vi "Turn Smother.vi"(2 "Ignore Deceleration":bool, 3 "Ignore Acceleration":bool, 4 "Internal Path Stuff":T2={"Trajectory Data"=[], "Updated Waypoints"=[], {"Sample Period (s)"=0.0, "Limits"={"Velocity (fps)"=0.0, "Accel (fps^2)"=0.0, "Jerk (fps^3)"=0.0, "StoopidFast (fps)"=0.0}, "Conditions"={"vInitial (fps)"=0.0, "vFinal (fps)"=0.0}, "Overrides"=[], "Angular Limits"={"Velocity (deg/s)"=6.0, "Accel (deg/s^2)"=15.0, "Jerk (deg/s^3)"=150.0}}, "Commands out"=[]} {"?"."Angular Limits"."Jerk (deg/s^3)" min=0.0 step=1.0; "?"."Angular Limits"."Accel (deg/s^2)" min=0.0; "?"."Angular Limits"."Velocity (deg/s)" min=0.0; "?"."Limits"."StoopidFast (fps)" min=0.0; "?"."Limits"."Jerk (fps^3)" min=0.0 step=1.0; "?"."Limits"."Accel (fps^2)" min=0.0; "?"."Limits"."Velocity (fps)" min=0.0; "?"."Overrides"."Angle Override" step=5.0; "?"."Overrides"."Velocity Override" step=5.0; "?"."Overrides"."Angular Override" step=5.0}) -> (1 "Overrides":T1 {"Angle Override" step=5.0; "Velocity Override" step=5.0; "Angular Override" step=5.0})   [LabVIEW 2023]
uses:
  Types/Internal Path Stuff.ctl
  Types/Trajectory Data.ctl
  Types/Segment Type.ctl
  Types/Limits.ctl
  Types/Overrides.ctl
  Types/Angluar Limits.ctl
  Types/Single Cmd Info.ctl
  <vilib>/picture/picture.llb/imagedata.ctl
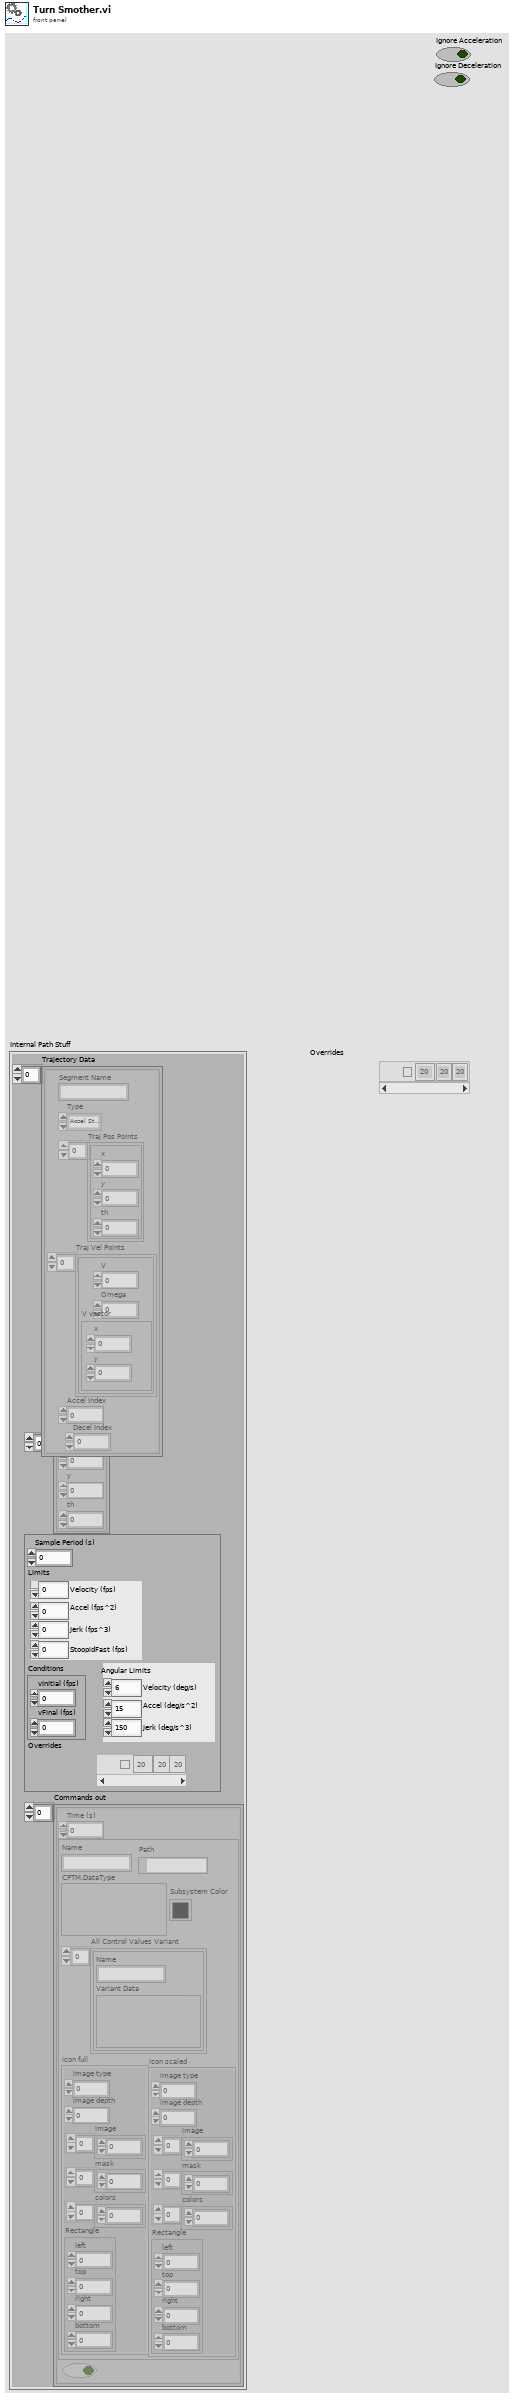
[diagram p1: front panel]
types:
  T1 = typedef "Overrides.ctl" = cluster{"Count":string, "Angular Override":dbl, "Enabled?":bool, "Velocity Override":dbl, "Angle Override":dbl}[]
  T2 = typedef "Internal Path Stuff.ctl" = cluster{"Trajectory Data":T3, "Updated Waypoints":cluster{"x":dbl, "y":dbl, "th":dbl}[], cluster{"Sample Period (s)":dbl, "Limits":T5, "Conditions":cluster{"vInitial (fps)":dbl, "vFinal (fps)":dbl}, "Overrides":T1, "Angular Limits":T6}, "Commands out":cluster{"Time (s)":dbl, T7, bool}[]}
  T3 = typedef "Trajectory Data.ctl" = cluster{"Segment Name":string, "Type":T4, "Traj Pos Points":cluster{"x":dbl, "y":dbl, "th":dbl}[], "Traj Vel Points":cluster{"V":dbl, "Omega":dbl, "V vector":cluster{"y":dbl, "x":dbl}}[], "Accel Index":i32, "Decel Index":i32}[]
  T4 = typedef "Segment Type.ctl" = enum16{"Accel Straight", "Const Straight", "Blend", "Circle", "Bezier"}
  T5 = typedef "Limits.ctl" = cluster{"Velocity (fps)":dbl, "Accel (fps^2)":dbl, "Jerk (fps^3)":dbl, "StoopidFast (fps)":dbl}
  T6 = typedef "Angluar Limits.ctl" = cluster{"Velocity (deg/s)":dbl, "Accel (deg/s^2)":dbl, "Jerk (deg/s^3)":dbl}
  T7 = typedef "Single Cmd Info.ctl" = cluster{"Name":string, "CPTM.DataType":variant, "All Control Values Variant":cluster{"Name":string, "Variant Data":variant}[], "icon full":T8, "icon scaled":T8, "Path":path, "Subsystem Color":u32}
  T8 = typedef "imagedata.ctl" = cluster{"image type":i32, "image depth":i32, "image":u8[], "mask":u8[], "colors":u32[], "Rectangle":cluster{"left":i16, "top":i16, "right":i16, "bottom":i16}}
  T9 = cluster{"Sample Period (s)":dbl, "Limits":T5, "Conditions":cluster{"vInitial (fps)":dbl, "vFinal (fps)":dbl}, "Overrides":T1, "Angular Limits":T6}
  T10 = cluster{"vInitial (fps)":dbl, "vFinal (fps)":dbl}
  T11 = cluster{string, dbl, bool, "Velocity (fps)":dbl, dbl}
  T12 = cluster{string, dbl, bool, "Velocity (fps)":dbl, dbl}[]
  T13 = cluster{"Segment Name":string, "Type":T4, "Traj Pos Points":cluster{"x":dbl, "y":dbl, "th":dbl}[], "Traj Vel Points":cluster{"V":dbl, "Omega":dbl, "V vector":cluster{"y":dbl, "x":dbl}}[], "Accel Index":i32, "Decel Index":i32}[]
  T14 = cluster{"Segment Name":string, "Type":T4, "Traj Pos Points":cluster{"x":dbl, "y":dbl, "th":dbl}[], "Traj Vel Points":cluster{"V":dbl, "Omega":dbl, "V vector":cluster{"y":dbl, "x":dbl}}[], "Accel Index":i32, "Decel Index":i32}
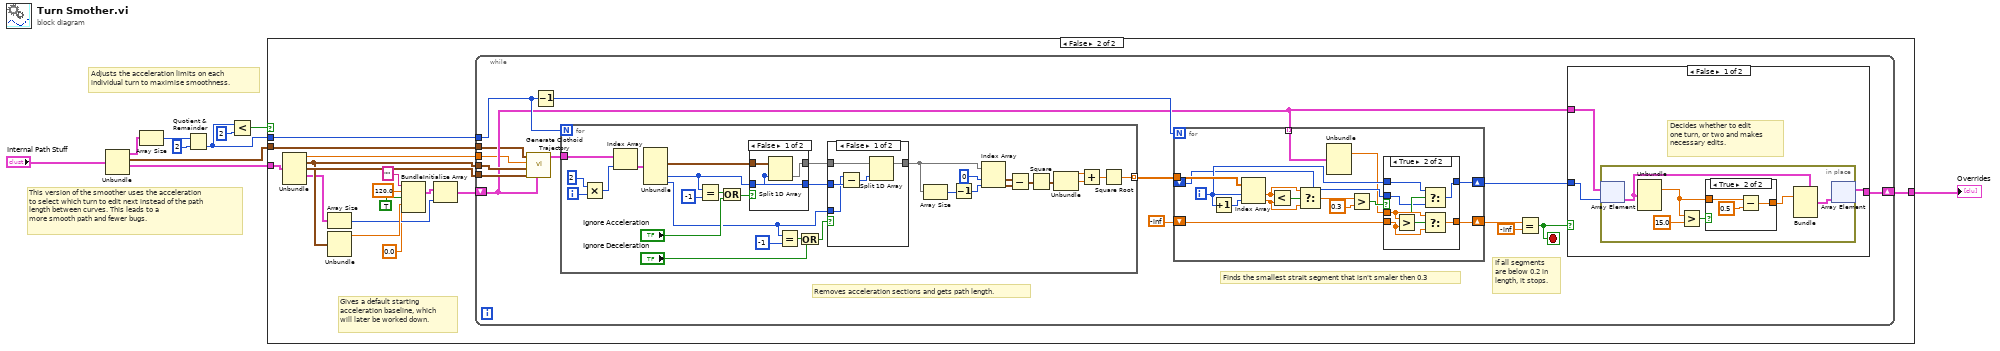
[diagram p0: block diagram]
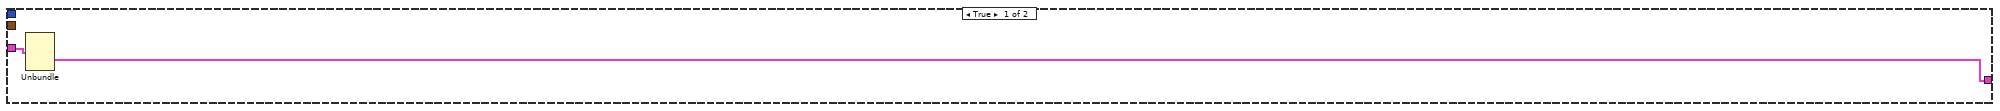
[diagram p2: hidden frame]
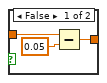
[diagram p3: hidden frame]
diagram:
  # "This version of the smoother uses the acceleration\nto select which turn to edit next instead of the path \nlength between curves. This leads to a \nmore smooth path and fewer bugs."
  # "Adjusts the acceleration limits on each \nindividual turn to maximise smoothness."
  n1 = Unbundle("Internal Path Stuff") -> ("Trajectory Data"=w4:T3, "Updated Waypoints"=w3:cluster{"x":dbl, "y":dbl, "th":dbl}[], w5:T9)  [unwired: 1 out]
  n2 = Array Size(array=w4) -> (size(s)=w10:i32)
  n3 = Quotient & Remainder(x=w10, y=2) -> (floor(x/y)=w7:i32)  [unwired: 1 out]
  n4 = Less?(x=w7, y=2) -> (x < y?=w6:bool)
  n5 = case shown="False" w6 {
    tunnel: w7 -> [_ w28]
    tunnel: [w12 w27] -> w2
    tunnel: w5 -> [w11 w26]
    tunnel: w3 -> [_ w24]
    frame True {
      n6 = Unbundle(w11) -> ("Overrides"=w12:T1)  [unwired: 4 out]
    }
    frame False {
      # "Gives a default starting \nacceleration baseline, which\nwill later be worked down."
      n7 = Unbundle(w26) -> ("Sample Period (s)"=w25:dbl, "Limits"=w22:T5, "Conditions"=w23:T10, "Overrides"=w21:T1)  [unwired: 1 out]
      n8 = Array Size(array=w21) -> (size(s)=w16:i32)
      n9 = Unbundle(w22) -> ("Velocity (fps)"=w17:dbl)  [unwired: 3 out]
      n10 = Bundle("", 120.0, TRUE, "Velocity (fps)"=w17, 0.0) -> (w15:T11)  [unwired: 1 in]
      n11 = Initialize Array(w15, w16) -> (w14:T12)
      n12 = while {
        shift-right: [w41] -> w27
        shift-left: w14 -> [w31]
        tunnel: w28 -> [w38]
        tunnel: w25 -> [w30]
        tunnel: w24 -> [w29]
        tunnel: w22 -> [w36]
        tunnel: w23 -> [w35]
        stop <- w43 stop-if-true
        # "If all segments\nare below 0.2 in\nlength, it stops."
        # "Removes acceleration sections and gets path length."
        # "Finds the smallest strait segment that isn't smaler then 0.3"
        n13 = call "Generate Clothoid Trajectory.vi"("Overrides"=w31, "Conditions"=w35, "Limits"=w36, "Sample Period (s)"=w30, "WayPoints"=w29) -> ("Trajectory Data Out"=w37:T13)  [unwired: 3 in, 3 out]
        n14 = Decrement(x=w38) -> (x-1=w39:i32)
        n15 = for {
          N: w38 -> [_]
          tunnel: w37 -> [w87]
          tunnel: [w77] -> w40 mode=indexing
          i -> [w89]
          n16 = Multiply(x=2, y=w89) -> (x*y=w86:i32)
          n17 = Index Array(array=w87, index=w86) -> (element=w85:T14)
          n18 = Unbundle(w85) -> ("Traj Pos Points"=w78:cluster{"x":dbl, "y":dbl, "th":dbl}[], "Accel Index"=w74:i32, "Decel Index"=w67:i32)  [unwired: 3 out]
          n19 = Equal?(x=w74, y=-1) -> (x = y?=w75:bool)
          n20 = Or(x=w75, y="Ignore Acceleration") -> (x .or. y?=w73:bool)
          n21 = case shown="False" w73 {
            tunnel: w78 -> [w98 w99]
            tunnel: [w97 w99] -> w84
            tunnel: [w96 _] -> w83
            tunnel: w74 -> [w96 _]
            frame False {
              n22 = Split 1D Array(array=w98, index=w96) -> (second subarray=w97:cluster{"x":dbl, "y":dbl, "th":dbl}[])  [unwired: 1 out]
            }
            frame True {
            }
          }
          n23 = Equal?(x=w67, y=-1) -> (x = y?=w70:bool)
          n24 = Or(x=w70, y="Ignore Deceleration") -> (x .or. y?=w68:bool)
          n25 = case shown="False" w68 {
            tunnel: w84 -> [w94 w95]
            tunnel: [w93 w95] -> w81
            tunnel: w83 -> [w92 _]
            tunnel: w67 -> [w90 _]
            frame False {
              n26 = Subtract(x=w90, y=w92) -> (x-y=w91:i32)
              n27 = Split 1D Array(array=w94, index=w91) -> (first subarray=w93:cluster{"x":dbl, "y":dbl, "th":dbl}[])  [unwired: 1 out]
            }
            frame True {
            }
          }
          n28 = Array Size(array=w81) -> (size(s)=w80:i32)
          n29 = Decrement(x=w80) -> (x-1=w79:i32)
          n30 = Index Array(array=w81, index #1=0 ("index"), index #2=w79) -> (element #1=w66:cluster{"x":dbl, "y":dbl, "th":dbl}, element #2=w65:cluster{"x":dbl, "y":dbl, "th":dbl})
          n31 = Subtract(x=w66, y=w65) -> (x-y=w64:cluster{"x":dbl, "y":dbl, "th":dbl})
          n32 = Square(x=w64) -> (x^2=w63:cluster{"x":dbl, "y":dbl, "th":dbl})
          n33 = Unbundle(w63) -> ("x"=w61:dbl, "y"=w62:dbl)  [unwired: 1 out]
          n34 = Add(x=w61, y=w62) -> (x+y=w60:dbl)
          n35 = Square Root(x=w60) -> (sqrt(x)=w77:dbl)
        }
        n36 = for {
          N: w39 -> [_]
          tunnel: w40 -> [w114]
          shift-right: [w109] -> w42
          shift-left: -inf -> [w108]
          tunnel: w31 -> [w101] mode=indexing
          shift-right: [w103] -> w32
          shift-left: _ -> [w102]
          i -> [w104]
          n37 = Increment(x=w104) -> (x+1=w113:i32)
          n38 = Index Array(array=w114, index #1=w104, index #2=w113) -> (element #1=w110:dbl, element #2=w111:dbl)
          n39 = Less?(x=w110, y=w111) -> (x < y?=w112:bool)
          n40 = Select(t=w110, s=w112, f=w111) -> (s? t:f=w106:dbl)
          n41 = Unbundle(w101) -> (w100:dbl)  [unwired: 4 out]
          n42 = Greater?(x=w106, y=0.3) -> (0:w107:bool)
          n43 = case shown="True" w107 {
            tunnel: [w116 w123] -> w109
            tunnel: w108 -> [w116 w122]
            tunnel: w100 -> [_ w121]
            tunnel: w104 -> [_ w119]
            tunnel: [w115 w117] -> w103
            tunnel: w102 -> [w115 w118]
            frame False {
            }
            frame True {
              n44 = Greater?(x=w121, y=w122) -> (0:w120:bool)
              n45 = Select(t=w119, s=w120, f=w118) -> (s? t:f=w117:i32)
              n46 = Select(t=w121, s=w120, f=w122) -> (s? t:f=w123:dbl)
            }
          }
        }
        n47 = Equal?(x=w42, y=-inf) -> (x = y?=w43:bool)
        n48 = case shown="False" w43 {
          tunnel: w31 -> [w44 w59]
          tunnel: [w45 w59] -> w41
          tunnel: w32 -> [w46 _]
          frame False {
            # "Decides whether to edit\none turn, or two and makes\nnecessary edits."
            n49 = in-place {
              n50 = in-place-array #1(w44, w46) -> (w49:T11)
              n51 = Unbundle(w49) -> (w50:dbl)  [unwired: 4 out]
              n52 = Greater?(x=w50, y=15.0) -> (0:w51:bool)
              n53 = case shown="True" w51 {
                tunnel: [w54 w57] -> w48
                tunnel: w50 -> [w55 w56]
                frame False {
                  n54 = Subtract(x=w55, y=0.05) -> (x-y=w54:dbl)
                }
                frame True {
                  n55 = Subtract(x=w56, y=0.5) -> (x-y=w57:dbl)
                }
              }
              n56 = Bundle(cluster=w49, w48) -> (w47:T11)  [unwired: 4 in]
              n57 = in-place-array #1(w47) -> (w45:T12)  [unwired: 1 out]
            }
          }
          frame True {
          }
        }
      }
    }
  }
  "Overrides" <- w2
